vi "Evaluate Step.vi"(0 "Step Config":T3, 1 "Plant Feedback":T2, 2 "Step Phase in":T1, 3 "step start ms":dbl, 4 "dwell start ms":dbl) -> (20 "Step Phase out":T1, 21 "dwell start ms out":dbl, 22 "done":bool, 23 "passed":bool, 24 "reason":string, 25 "measured":dbl, 26 "target":dbl)   [LabVIEW 2026]
doc: "Evaluates the active step on one feedback sample; now is the feedback's timestamp_ms. Idle or Complete in: unchanged, done FALSE. Settling: timeout (now - step start >= timeout_ms) gives Complete, done, not passed, reason Timeout; else within tolerance gives Dwell with dwell start out = now. Dwell: timeout first (as above); else out of tolerance gives Settling; else (now - dwell start) >= dwell_time_ms gives Complete, done, passed, reason empty. An unknown monitored_io gives Complete, done, not passed, reason Unknown monitored IO. measured and target are always output. Pure function, no error terminals, AF-free."
uses:
  Typedefs/Step Config.ctl
  Typedefs/Plant Feedback.ctl
  Typedefs/Step Phase.ctl
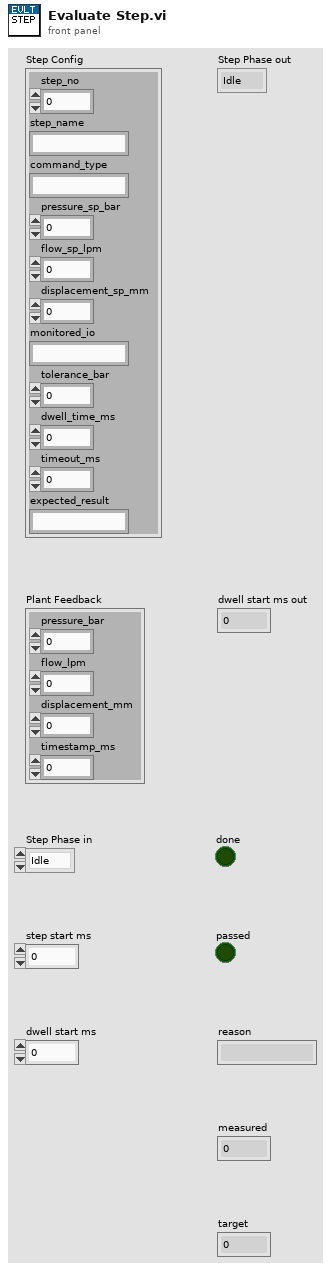
[diagram p1: front panel]
types:
  T1 = typedef "Step Phase.ctl" = enum16{"Idle", "Settling", "Dwell", "Complete"}
  T2 = typedef "Plant Feedback.ctl" = cluster{"pressure_bar":dbl, "flow_lpm":dbl, "displacement_mm":dbl, "timestamp_ms":dbl}
  T3 = typedef "Step Config.ctl" = cluster{"step_no":i32, "step_name":string, "command_type":string, "pressure_sp_bar":dbl, "flow_sp_lpm":dbl, "displacement_sp_mm":dbl, "monitored_io":string, "tolerance_bar":dbl, "dwell_time_ms":i32, "timeout_ms":i32, "expected_result":string}
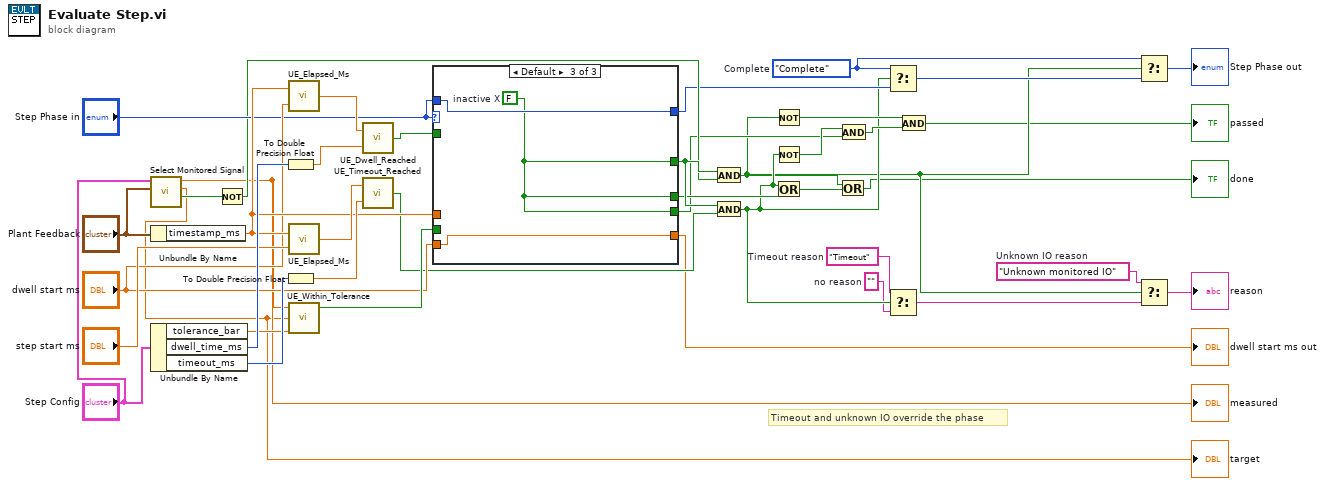
[diagram p0: block diagram]
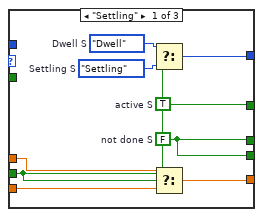
[diagram p2: hidden frame]
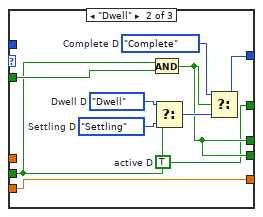
[diagram p3: hidden frame]
diagram:
  w9 = "Unknown monitored IO"  # Unknown IO reason
  w11 = ""  # no reason
  w12 = "Timeout"  # Timeout reason
  w21 = Step_Phase."Complete"  # Complete
  # "Timeout and unknown IO override the phase"
  n1 = call "Select Monitored Signal.vi"("Plant Feedback"="Plant Feedback", "Step Config"="Step Config") -> ("valid"=w25:bool, "target"=w1:dbl, "measured"=w2:dbl)  [unwired: 7 in]
  "measured" <- w2
  "target" <- w1
  n2 = Unbundle By Name("Plant Feedback") -> ("timestamp_ms"=w29:dbl)
  n3 = Unbundle By Name("Step Config") -> ("tolerance_bar"=w34:dbl, "dwell_time_ms"=w39:i32, "timeout_ms"=w38:i32)
  n4 = Not(x=w25) -> (.not. x?=w23:bool)
  n5 = To Double Precision Float(number=w39) -> (double precision float=w32:dbl)
  n6 = To Double Precision Float(number=w38) -> (double precision float=w35:dbl)
  n7 = call "UE_Elapsed_Ms.vi"("start_ms"="dwell start ms", "now_ms"=w29) -> ("elapsed_ms"=w33:dbl)
  n8 = call "UE_Elapsed_Ms.vi"("start_ms"="step start ms", "now_ms"=w29) -> ("elapsed_ms"=w36:dbl)
  n9 = call "UE_Within_Tolerance.vi"("tolerance"=w34, "target"=w1, "actual"=w2) -> ("within_tolerance"=w31:bool)  [unwired: 2 in]
  n10 = call "UE_Dwell_Reached.vi"("threshold_ms"=w32, "elapsed_ms"=w33) -> ("reached"=w30:bool)
  n11 = call "UE_Timeout_Reached.vi"("threshold_ms"=w35, "elapsed_ms"=w36) -> ("reached"=w26:bool)
  n12 = case shown="Default" "Step Phase in" {
    tunnel: "Step Phase in" -> [_ _ w63]
    tunnel: w31 -> [w48 w59 _]
    tunnel: w30 -> [_ w60 _]
    tunnel: w29 -> [w47 _ _]
    tunnel: "dwell start ms" -> [w46 w52 w62]
    tunnel: [w45 w54 w63] -> w22
    tunnel: [w44 w53 w61] -> w19
    tunnel: [w44 w53 w61] -> w16
    tunnel: [w43 w52 w62] -> w6
    tunnel: [w42 w51 w61] -> w24
    frame "Settling" {
      w42 = TRUE  # active S
      w44 = FALSE  # not done S
      w49 = Step_Phase."Settling"  # Settling S
      w50 = Step_Phase."Dwell"  # Dwell S
      n13 = Select(t=w50, s=w48, f=w49) -> (s? t:f=w45:T1)
      n14 = Select(t=w47, s=w48, f=w46) -> (s? t:f=w43:dbl)
    }
    frame "Dwell" {
      w51 = TRUE  # active D
      w56 = Step_Phase."Complete"  # Complete D
      w57 = Step_Phase."Settling"  # Settling D
      w58 = Step_Phase."Dwell"  # Dwell D
      n15 = And(x=w59, y=w60) -> (x .and. y?=w53:bool)
      n16 = Select(t=w58, s=w59, f=w57) -> (s? t:f=w55:T1)
      n17 = Select(t=w56, s=w53, f=w55) -> (s? t:f=w54:T1)
    }
    frame Default {
      w61 = FALSE  # inactive X
    }
  }
  "dwell start ms out" <- w6
  n18 = And(x=w24, y=w23) -> (x .and. y?=w10:bool)
  n19 = And(x=w24, y=w26) -> (x .and. y?=w13:bool)
  n20 = Not(x=w10) -> (.not. x?=w15:bool)
  n21 = Not(x=w13) -> (.not. x?=w17:bool)
  n22 = Or(x=w13, y=w19) -> (x .or. y?=w18:bool)
  n23 = Or(x=w10, y=w18) -> (x .or. y?=→"done":bool)
  n24 = And(x=w17, y=w16) -> (x .and. y?=w14:bool)
  n25 = Select(t=w21, s=w13, f=w22) -> (s? t:f=w20:T1)
  n26 = Select(t=w12, s=w13, f=w11) -> (s? t:f=w8:string)
  n27 = And(x=w15, y=w14) -> (x .and. y?=→"passed":bool)
  n28 = Select(t=w21, s=w10, f=w20) -> (s? t:f=→"Step Phase out":T1)
  n29 = Select(t=w9, s=w10, f=w8) -> (s? t:f=→"reason":string)
